vi "test prompts list required.vi"(8 "error in (no error)":errorcluster) -> (0 "error out":errorcluster, 3 "body":string)   [LabVIEW 2020, in "MCP Server tests.lvlib"]
doc: "Every argument in prompts/list has required true or false, taken from the connector pane of the prompt VI."
uses:
  MCP Server tests.lvlib
  <vilib>/addons/_JKI Toolkits/Caraya/classes/Test/Test.lvclass
  <vilib>/addons/_JKI Toolkits/Caraya/classes/Assert/Assert.lvclass
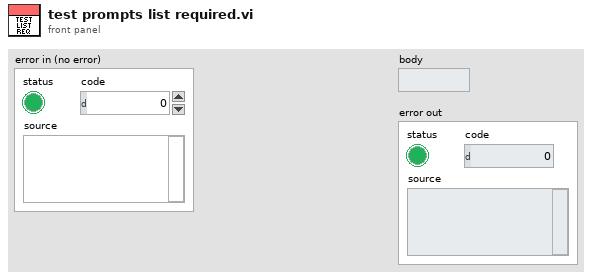
[diagram p1: front panel]
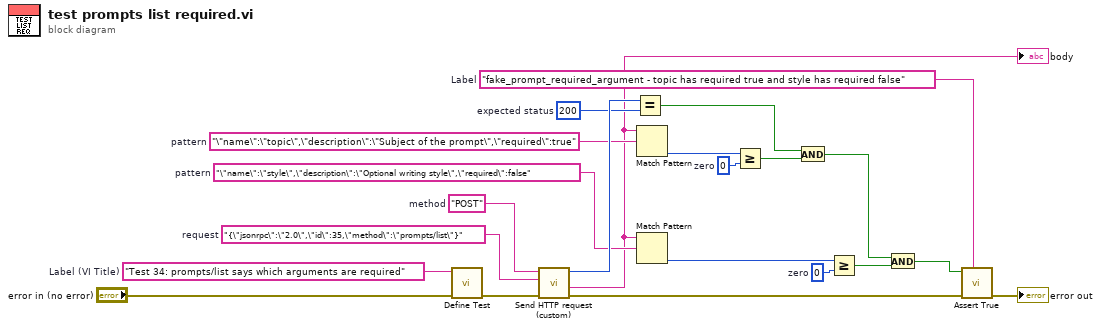
[diagram p0: block diagram]
diagram:
  w3 = "fake_prompt_required_argument - topic has required true and style has required false"  # Label
  w10 = 0  # zero
  w12 = "\"name\":\"style\",\"description\":\"Optional writing style\",\"required\":false"  # pattern
  w13 = 0  # zero
  w15 = "\"name\":\"topic\",\"description\":\"Subject of the prompt\",\"required\":true"  # pattern
  w16 = 200  # expected status
  w19 = "{\"jsonrpc\":\"2.0\",\"id\":35,\"method\":\"prompts/list\"}"  # request
  w20 = "POST"  # method
  w22 = "Test 34: prompts/list says which arguments are required"  # Label (VI Title)
  n1 = call <vilib>:"Define Test.vi"("error in (no error)"="error in (no error)", "Label (VI Title)"=w22) -> ("error out"=w18:errorcluster)  [unwired: 8 in, 1 out]
  n2 = call "Send HTTP request (custom).vi"("error in (no error)"=w18, "request"=w19, "method"=w20) -> ("error out"=w4:errorcluster, "response"=w2:string, "status code"=w17:i32)  [unwired: 5 in, 1 out]
  "body" <- w2
  n3 = Equal?(x=w17, y=w16) -> (x = y?=w9:bool)
  n4 = Match Pattern(string=w2, regular expression=w15) -> (offset past match=w14:i32)  [unwired: 1 in, 3 out]
  n5 = Match Pattern(string=w2, regular expression=w12) -> (offset past match=w11:i32)  [unwired: 1 in, 3 out]
  n6 = Greater Or Equal?(x=w14, y=w13) -> (x >= y?=w8:bool)
  n7 = And(x=w9, y=w8) -> (x .and. y?=w7:bool)
  n8 = Greater Or Equal?(x=w11, y=w10) -> (x >= y?=w6:bool)
  n9 = And(x=w7, y=w6) -> (x .and. y?=w5:bool)
  n10 = call <vilib>:"Assert True.vi"("Label"=w3, "error in (no error)"=w4, "True?"=w5) -> ("error out"=→"error out":errorcluster)  [unwired: 7 in, 1 out]
